vi "_caraya_updateVInames.vi"(8 "error in (no error)":errorcluster, 10 "Application":refnum<vi>, 11 "Class Path":path=path "C:/Projects/JKI/Caraya/src/tests/test-all-asserts/Test Runner.AllAsserts.lvclass") -> (0 "error out":errorcluster)   [LabVIEW 2020]
uses:
  <vilib>/regexp/Match Regular Expression.xnode
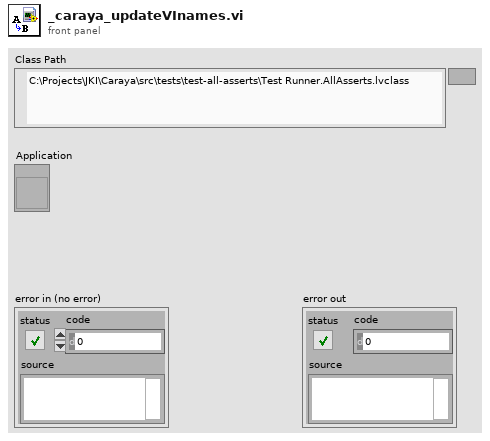
[diagram p1: front panel]
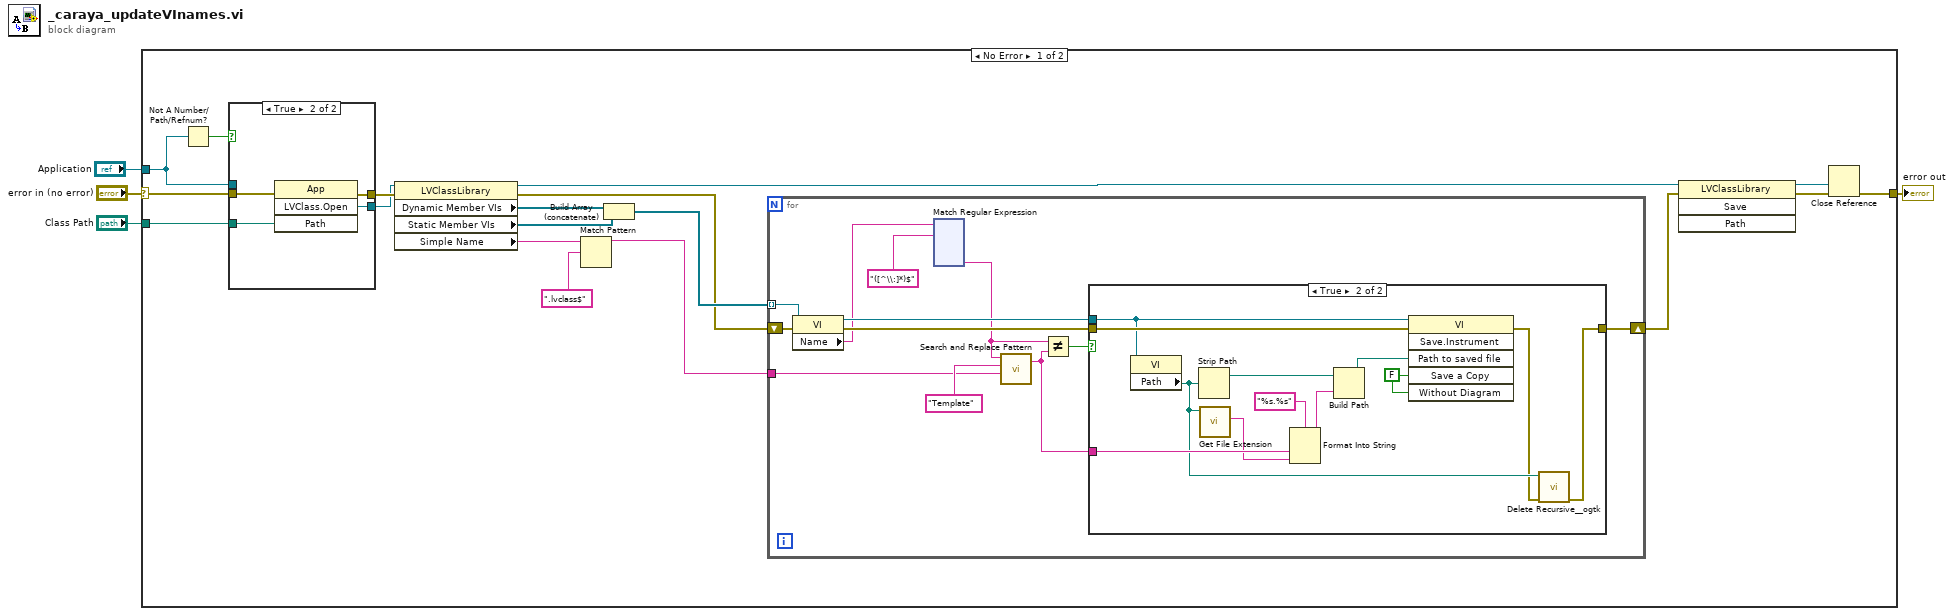
[diagram p0: block diagram]
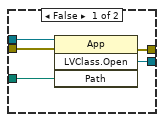
[diagram p2: hidden frame]
diagram:
  n1 = case shown="No Error" "error in (no error)" {
    selector: "error in (no error)" -> [w5 w173]
    tunnel: "Class Path" -> [w14 _]
    tunnel: [w11 w173] -> w3
    tunnel: "Application" -> [w10 _]
    frame No Error {
      n2 = Not A Number/Path/Refnum?(number/path/refnum=w10) -> (NaN/Path/Refnum?=w9:bool)
      n3 = case shown="True" w9 {
        tunnel: [w27 w31] -> w17
        tunnel: [w26 w30] -> w15
        tunnel: w14 -> [w25 w29]
        tunnel: w5 -> [w24 w28]
        tunnel: w10 -> [w23 _]
        frame False {
          n4 = invoke class="App" method="LVClass.Open"(reference=w23, error in=w24, "Path"=w25) -> (error out=w27:errorcluster, "LVClass.Open"=w26:refnum<vi>)  [unwired: 1 in, 2 out]
        }
        frame True {
          n5 = invoke class="App" method="LVClass.Open"(error in=w28, "Path"=w29) -> (error out=w31:errorcluster, "LVClass.Open"=w30:refnum<vi>)  [unwired: 2 in, 2 out]
        }
      }
      n6 = property class="LVClassLibrary"(reference=w15, error in=w17) -> (reference out=w16:refnum<vi>, error out=w13:errorcluster, "Dynamic Member VIs"=w22:refnum<vi>[], "Static Member VIs"=w21:refnum<vi>[], "Simple Name"=w7:string)
      n7 = Match Pattern(string=w7, regular expression=".lvclass$") -> (before substring=w6:string)  [unwired: 1 in, 3 out]
      n8 = Build Array (concatenate)(w22, w21) -> (w20:refnum<vi>[])
      n9 = for {
        tunnel: w20 -> [w36] mode=indexing
        shift-right: [w39] -> w12
        shift-left: w13 -> [w37]
        tunnel: w6 -> [w42]
        n10 = property class="VI"(reference=w36, error in=w37) -> (reference out=w40:refnum<vi>, error out=w38:errorcluster, "Name"=w34:string)
        n11 = xnode "Match Regular Expression"("input string"=w34, "regular expression"="([^\\:]*)$") -> ("submatch 1"=w33:string)  [unwired: 4 in, 5 out]
        n12 = call <vilib>:"Search and Replace Pattern.vi"("string"=w33, "regular expression (\"\")"="Template" ("regular expression"), "replace string (\"\")"=w42) -> ("result string"=w41:string)  [unwired: 2 in, 1 out]
        n13 = Not Equal?(x=w33, y=w41) -> (x != y?=w32:bool)
        n14 = case shown="True" w32 {
          tunnel: w40 -> [_ w171]
          tunnel: w41 -> [_ w169]
          tunnel: w38 -> [w160 w172]
          tunnel: [w160 w161] -> w39
          frame False {
          }
          frame True {
            w164 = FALSE ("Save a Copy")
            n15 = property class="VI"(reference=w171) -> ("Path"=w163:path)  [unwired: 1 in, 2 out]
            n16 = Strip Path(path=w163) -> (stripped path=w170:path)  [unwired: 1 out]
            n17 = call <vilib>:"Get File Extension.vi"("file"=w163) -> ("lowercase file extension"=w168:string)  [unwired: 6 in, 4 out]
            n18 = Format Into String(format string="%s.%s", w169, w168) -> (resulting string=w166:string)  [unwired: 2 in, 1 out]
            n19 = Build Path(base path=w170, name or relative path=w166) -> (appended path=w165:path)
            n20 = invoke class="VI" method="Save.Instrument"(reference=w171, error in=w172, "Path to saved file"=w165, "Save a Copy"=w164, "Without Diagram"=w164) -> (error out=w162:errorcluster)  [unwired: 1 in, 5 out]
            n21 = call <userlib>:"Delete Recursive__ogtk.vi"("error in (no error)"=w162, "Path"=w163) -> ("error out"=w161:errorcluster)  [unwired: 8 in, 1 out]
          }
        }
      }
      n22 = invoke class="LVClassLibrary" method="Save"(reference=w16, error in=w12) -> (reference out=w18:refnum<vi>, error out=w19:errorcluster)  [unwired: 2 in, 2 out]
      n23 = Close Reference(reference=w18, error in (no error)=w19) -> (error out=w11:errorcluster)
    }
    frame Error {
    }
  }
  "error out" <- w3
